vi "Start Writer.vi"(8 "error in (no error)":errorcluster, 11 "XNET_CAN_RW in":refnum<class "XNET CAN RW.lvclass">) -> (0 "error out":errorcluster, 3 "XNET_CAN_RW out":refnum<class "XNET CAN RW.lvclass">)   [LabVIEW 2021, in "XNET CAN RW.lvclass"]
uses:
  XNET CAN RW.lvclass
  C:/Program Files/National Instruments/LabVIEW 2021/vi.lib/CIF Foundation/CIF CAN RW Core/CAN_RW_CORE.lvclass
  <vilib>/CIF Foundation/CIF CAN RW Core/CAN_RW_CORE.lvclass/CAN_RW_CORE.ctl
  <vilib>/CIF Foundation/CIF CAN RW Core/typedef/CAN Interface Mode.ctl
  XNET CAN RW.lvclass/XNET CAN RW.ctl
  <vilib>/CIF Foundation/CIF CAN RW Core/Accessors/Read Interface.vi
  <vilib>/CIF Foundation/CIF CAN RW Core/Accessors/Read Port Configuration.vi
  <vilib>/CIF Foundation/CIF CAN RW Core/Accessors/Write CAN Interface Mode.vi
  <vilib>/xnet/xnet.llb/XNET Create Session (Frame Output Stream).vi
  <resource>/objmgr/xnet.rc
  <vilib>/CIF Foundation/CIF CAN RW Core/CAN_RW_CORE.lvclass
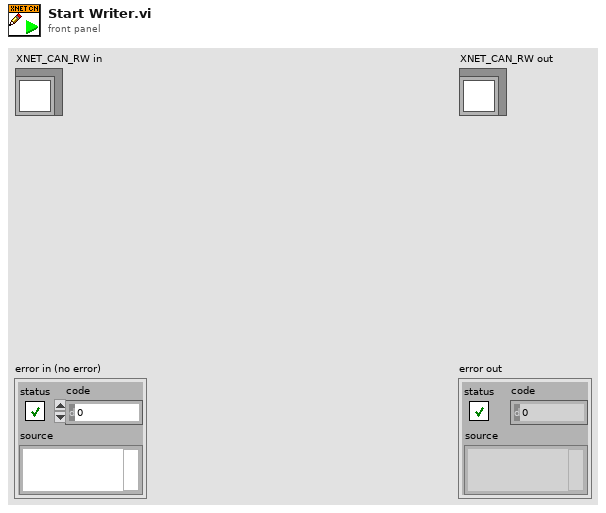
[diagram p1: front panel]
types:
  T1 = typedef "CAN_RW_CORE.lvclass/CAN Port Configuration.ctl" = cluster{"Mode":T2, "Baud Rate":u64, "Temination On":bool, "Subordinate":bool, "Echo TX":bool, "FD Config":T3}
  T2 = typedef "CAN_RW_CORE.lvclass/CAN Mode.ctl" = enum16{"CAN 2.0", "CAN FD"}
  T3 = typedef "CAN_RW_CORE.lvclass/FD Config.ctl" = cluster{"FD Baud Rate":u64, "ISO Mode":bool, "BRS Enabled":bool}
  T4 = typedef "CAN_RW_CORE.lvclass/CAN Interface Mode.ctl" = enum16{"Unknown", "CAN 2.0", "CAN FD", "CAN FD BRS"}
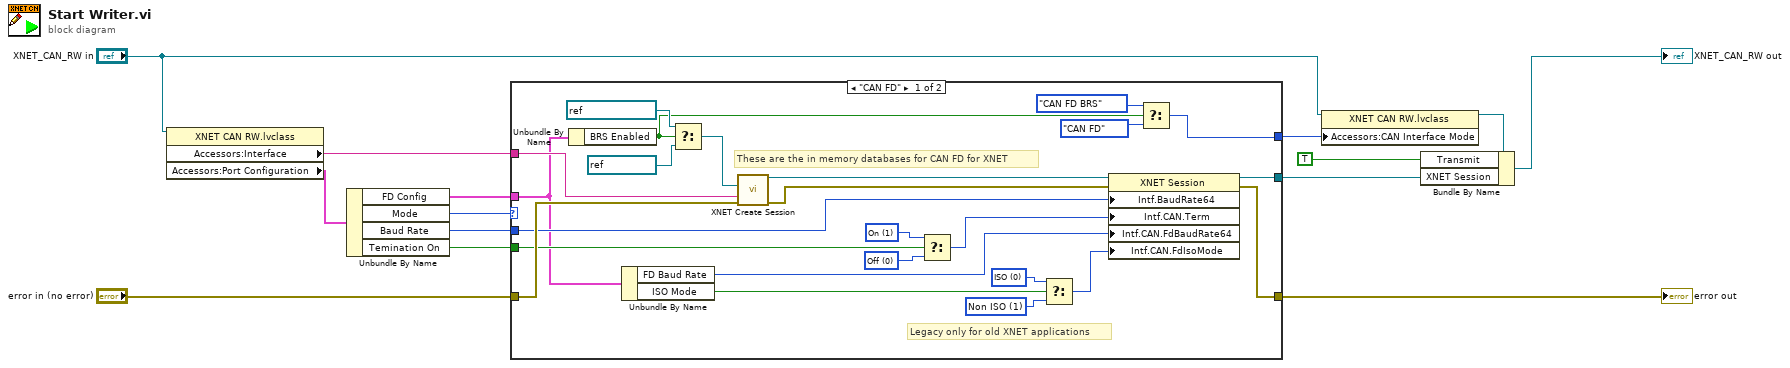
[diagram p0: block diagram]
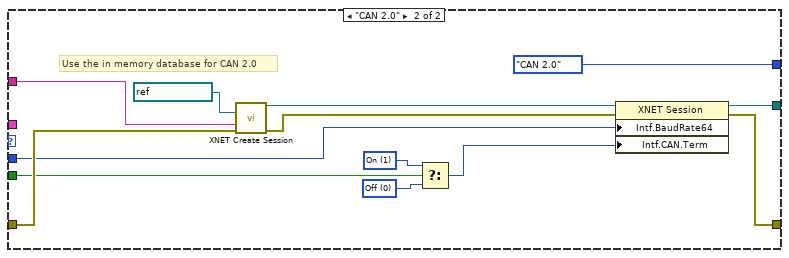
[diagram p2: hidden frame]
diagram:
  n1 = property class="XNET CAN RW.lvclass"(reference="XNET_CAN_RW in") -> ("Accessors:Interface"=w4:string, "Accessors:Port Configuration"=w5:T1)  [unwired: 1 in, 2 out]
  n2 = Unbundle By Name(w5) -> ("FD Config"=w12:T3, "Mode"=w11:T2, "Baud Rate"=w13:u64, "Temination On"=w7:bool)
  n3 = case shown="\"CAN FD\"" w11 {
    tunnel: w4 -> [w38 w51]
    tunnel: "error in (no error)" -> [w37 w50]
    tunnel: w13 -> [w29 w45]
    tunnel: w7 -> [w30 w46]
    tunnel: w12 -> [w27 _]
    tunnel: [w22 w43] -> w8
    tunnel: [w21 w42] -> w9
    tunnel: [w15 CAN_Interface_Mode."CAN 2.0" ("CAN Interface Mode")] -> w3
    frame "CAN FD" {
      w24 = u32 1 items=["ISO", "Non ISO", "ISO Legacy"] ("Interface:CAN:FD ISO Mode")
      w25 = u32 0 items=["ISO", "Non ISO", "ISO Legacy"] ("Interface:CAN:FD ISO Mode")
      w28 = u32 0 items=["Off", "On"] ("Interface:CAN:Termination")
      w32 = u32 1 items=["Off", "On"] ("Interface:CAN:Termination")
      # "These are the in memory databases for CAN FD for XNET"
      # "Legacy only for old XNET applications"
      n4 = Unbundle By Name(w27) -> ("BRS Enabled"=w16:bool)
      n5 = Unbundle By Name(w27) -> ("FD Baud Rate"=w20:u64, "ISO Mode"=w26:bool)
      n6 = Select(t=refnum<k21> ":can_fd_brs:" ("cluster (:memory:)"), s=w16, f=refnum<k21> ":can_fd:" ("cluster (:memory:)")) -> (s? t:f=w34:refnum<k21>)
      n7 = call-poly <vilib>:"XNET Create Session.vi"("cluster (:memory:)"=w34, "interface"=w38, "error in (no error)"=w37) -> ("session out"=w33:refnum<k21>, "error out"=w31:errorcluster)  [unwired: 11 in]
      n8 = Select(t=w32, s=w30, f=w28) -> (s? t:f=w19:u32)
      n9 = Select(t=w25, s=w26, f=w24) -> (s? t:f=w23:u32)
      n10 = property class="XNET Session"(reference=w33, error in=w31, "Intf.BaudRate64"=w29, "Intf.CAN.Term"=w19, "Intf.CAN.FdBaudRate64"=w20, "Intf.CAN.FdIsoMode"=w23) -> (reference out=w21:refnum<k21>, error out=w22:errorcluster)
      n11 = Select(t=CAN_Interface_Mode."CAN FD BRS" ("CAN Interface Mode"), s=w16, f=CAN_Interface_Mode."CAN FD" ("CAN Interface Mode")) -> (s? t:f=w15:T4)
    }
    frame "CAN 2.0" {
      w44 = u32 0 items=["Off", "On"] ("Interface:CAN:Termination")
      w48 = u32 1 items=["Off", "On"] ("Interface:CAN:Termination")
      # "Use the in memory database for CAN 2.0"
      n12 = call-poly <vilib>:"XNET Create Session.vi"("cluster (:memory:)"=refnum<k21> ":memory:", "interface"=w51, "error in (no error)"=w50) -> ("session out"=w49:refnum<k21>, "error out"=w47:errorcluster)  [unwired: 11 in]
      n13 = Select(t=w48, s=w46, f=w44) -> (s? t:f=w41:u32)
      n14 = property class="XNET Session"(reference=w49, error in=w47, "Intf.BaudRate64"=w45, "Intf.CAN.Term"=w41) -> (reference out=w42:refnum<k21>, error out=w43:errorcluster)
    }
  }
  "error out" <- w8
  n15 = property class="XNET CAN RW.lvclass"(reference="XNET_CAN_RW in", "Accessors:CAN Interface Mode"=w3) -> (reference out=w1:refnum<class "XNET CAN RW.lvclass">)  [unwired: 1 in, 1 out]
  n16 = Bundle By Name(cluster=w1, "Transmit"=TRUE, "XNET Session"=w9) -> (→"XNET_CAN_RW out":refnum<class "XNET CAN RW.lvclass">)
